vi "Digital_Write_Ex.vi"() -> ()   [LabVIEW 2026]
panel:
  in  "VISA resource name":refnum<visa-resource-name>
  in  "Stop Button":bool
  out "respuesta":string
  out "error out":errorcluster
  in  "Canal":u8
  in  "Valor":bool
  # "Ejemplo: Digital Write"
  # "Descripción: pone en alto o en bajo una salida digital."
  # "Configuracion"
  # "Indicadores"
  # "Control"
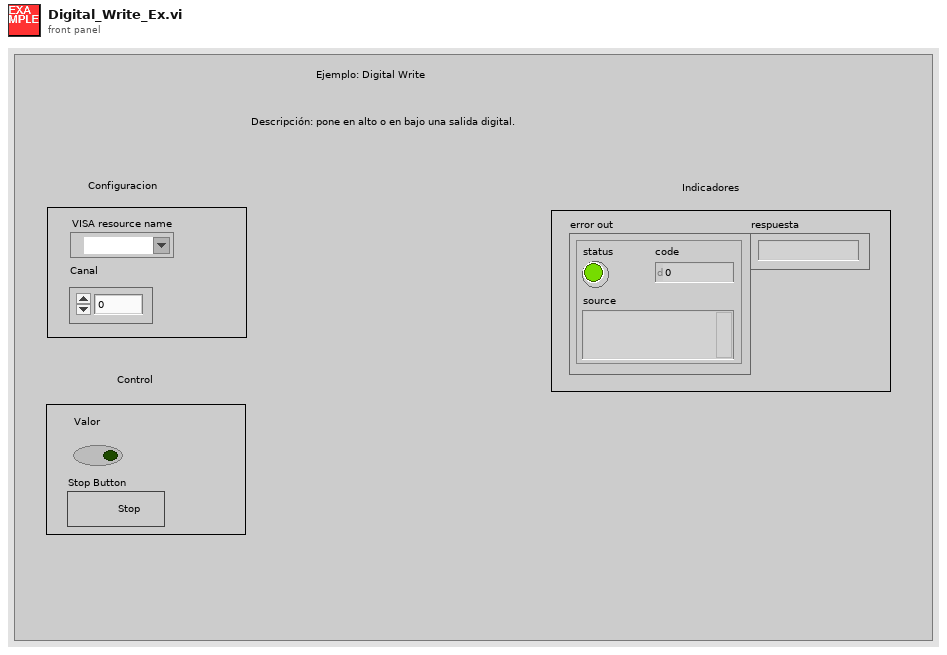
[diagram p1: front panel]
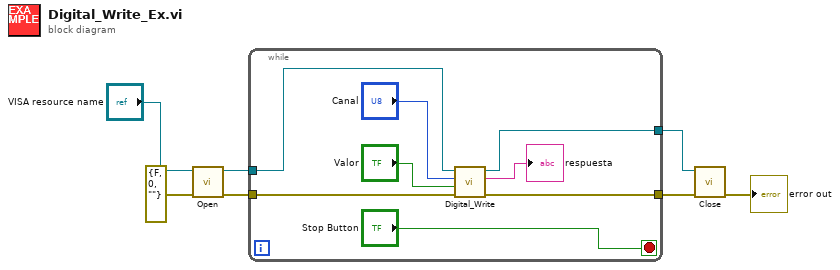
[diagram p0: block diagram]
diagram:
  n1 = call "Open.vi"("error in (no error)"=errorcluster {"status"=FALSE, "code"=0, "source"=""}, "VISA resource name"="VISA resource name") -> ("error out"=w7:errorcluster, "VISA resource name out"=w6:refnum<visa-resource-name>)  [unwired: 8 in]
  n2 = while {
    tunnel: w6 -> [w12]
    tunnel: [w9] -> w5
    tunnel: w7 -> [w15]
    tunnel: [w11] -> w4
    stop <- "Stop Button" stop-if-true
    n3 = call "Digital_Write.vi"("error in (no error)"=w15, "Valor"="Valor", "Canal"="Canal", "VISA resource name"=w12) -> ("error out"=w11:errorcluster, "respuesta"=→"respuesta":string, "VISA resource name out"=w9:refnum<visa-resource-name>)  [unwired: 5 in]
  }
  n4 = call "Close.vi"("error in (no error)"=w4, "VISA resource name"=w5) -> ("error out"=→"error out":errorcluster)  [unwired: 9 in]
